vi "Layout.vi"(0 "reference":refnum<class "ClassRelationshipEdge.lvclass">, 1 "graph":refnum<class "Graph.lvclass">, 2 "graphics":refnum<class "Graphics.lvclass">, 3 "grid":refnum<class "Grid.lvclass">, 5 "error in (no error)":errorcluster) -> (14 "reference out":refnum<class "ClassRelationshipEdge.lvclass">, 19 "error out":errorcluster)   [LabVIEW 2020, in "ClassRelationshipEdge.lvclass"]
uses:
  <resource>/Framework/Providers/Open_GDS/UML/ClassRelationshipEdge_class/ClassRelationshipEdge.lvclass
  C:/Program Files (x86)/National Instruments/LabVIEW 2020/resource/Framework/Providers/Open_GDS/UML/AbstractEdge_class/AbstractEdge.lvclass
  <resource>/Framework/Providers/Open_GDS/UML/Grid_class/Grid.lvclass
  <resource>/Framework/Providers/Open_GDS/UML/Graphics_class/Graphics.lvclass
  <resource>/Framework/Providers/Open_GDS/UML/Graph_class/Graph.lvclass
  <resource>/Framework/Providers/Open_GDS/UML/BentStyle_class/BentStyle.lvclass
  <resource>/Framework/Providers/Open_GDS/UML/AbstractNode_class/AbstractNode.lvclass
  <resource>/Framework/Providers/Open_GDS/UML/AbstractEdge_class/AbstractEdge.lvclass
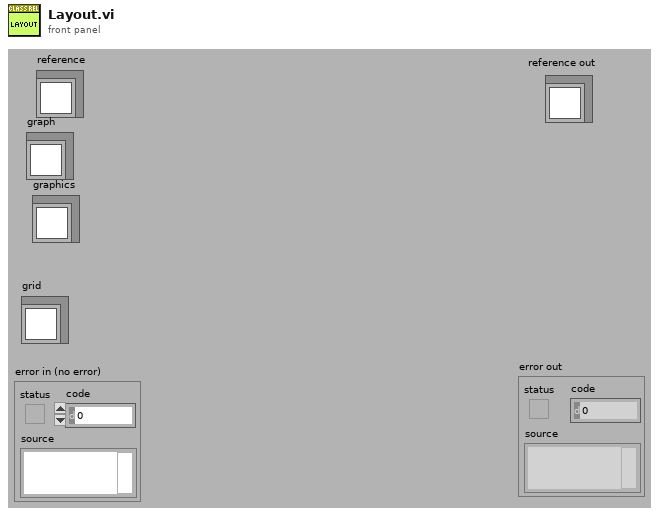
[diagram p1: front panel]
types:
  T1 = typedef "ClassRelationshipEdge.lvclass/ObjectAttributes.ctl" = cluster{"bentStyleRef":refnum<class "BentStyle.lvclass">, "startConnectionOffset":cluster{"x":i32, "y":i32}, "endConnectionOffset":cluster{"x":i32, "y":i32}, "MidLineOffset":cluster{"x":i32, "y":i32}, "DepClass":T2}
  T2 = typedef "ReversedEngineering_ViDependencyDetailsType.ctl" = cluster{"ThisVIs/Ctls":path[], "Dependent_VIs/Ctls":path[]}
  T3 = typedef "AbstractEdge.lvclass/ObjectAttributes.ctl" = cluster{"start":refnum<class "AbstractNode.lvclass">, "end":refnum<class "AbstractNode.lvclass">}
  T4 = typedef "Rectangle Rectangle2D.ctl" = cluster{"x":dbl, "y":dbl, "width":dbl, "height":dbl}
  T5 = typedef "Point Point2D.ctl" = cluster{"x":dbl, "y":dbl}
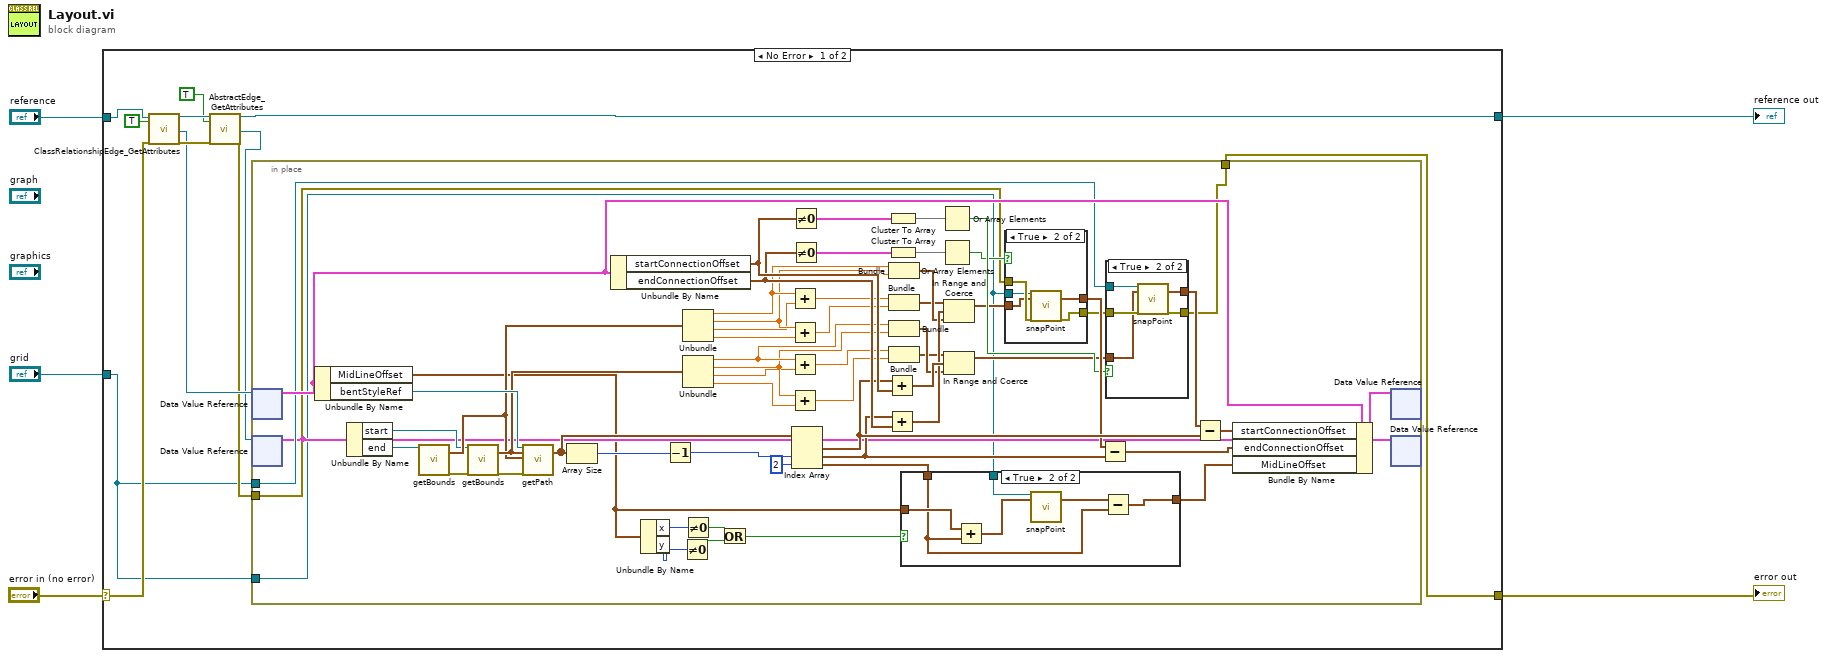
[diagram p0: block diagram]
diagram:
  n1 = case shown="No Error" "error in (no error)" {
    selector: "error in (no error)" -> [w17 w100]
    tunnel: "reference" -> [w16 w101]
    tunnel: [w15 w100] -> w3
    tunnel: [w14 w101] -> w2
    tunnel: "grid" -> [w7 _]
    frame No Error {
      n2 = call <resource>:"ClassRelationshipEdge_GetAttributes.vi"("reference in"=w16, "OnlyGetDvrReference(False)"=TRUE, "error in (no error)"=w17) -> ("reference out"=w12:refnum<class "ClassRelationshipEdge.lvclass">, "DataRef"=w10:refnum<data-value>, "error out"=w11:errorcluster)  [unwired: 13 in, 1 out]
      n3 = call <resource>:"AbstractEdge_GetAttributes.vi"("reference in"=w12, "OnlyGetDvrReference(False)"=TRUE, "error in (no error)"=w11) -> ("reference out"=w14:refnum<class "ClassRelationshipEdge.lvclass">, "DataRef"=w9:refnum<data-value>, "error out"=w8:errorcluster)  [unwired: 13 in, 1 out]
      n4 = in-place {
        in-place-border: w7 -> [w56]
        in-place-border: [w55] -> w15
        in-place-border: w8 -> [w53]
        in-place-border: w7 -> [w27]
        n5 = in-place-dvr #1(w10) -> (w78:T1)  [unwired: 1 out]
        n6 = in-place-dvr #2(w9) -> (w28:T3)  [unwired: 1 out]
        n7 = Unbundle By Name(w78) -> ("MidLineOffset"=w20:cluster{"x":i32, "y":i32}, "bentStyleRef"=w75:refnum<class "BentStyle.lvclass">)
        n8 = Unbundle By Name(w28) -> ("start"=w51:refnum<class "AbstractNode.lvclass">, "end"=w45:refnum<class "AbstractNode.lvclass">)
        n9 = call-dynamic "getBounds.vi"("reference"=w45) -> ("bounds"=w67:T4, "error out"=w50:errorcluster)  [unwired: 1 in, 16 out]
        n10 = call-dynamic "getBounds.vi"("reference"=w51, "error in (no error)"=w50) -> ("bounds"=w68:T4, "error out"=w66:errorcluster)  [unwired: 16 out]
        n11 = call-dynamic "getPath.vi"("reference"=w75, "start"=w68, "end"=w67, "error in (no error)"=w66) -> ("path"=w65:T5[])  [unwired: 15 out]
        n12 = Array Size(array=w65) -> (size(s)=w40:i32)
        n13 = Unbundle By Name(w78) -> ("startConnectionOffset"=w74:cluster{"x":i32, "y":i32}, "endConnectionOffset"=w73:cluster{"x":i32, "y":i32})
        n14 = Unbundle By Name(w20) -> ("x"=w24:i32, "y"=w23:i32)
        n15 = Decrement(x=w40) -> (x-1=w60:i32)
        n16 = Not Equal To 0?(x=w23) -> (x != 0?=w21:bool)
        n17 = Unbundle(w67) -> ("x"=w44:dbl, "y"=w43:dbl, "width"=w42:dbl, "height"=w41:dbl)
        n18 = Unbundle(w68) -> ("x"=w49:dbl, "y"=w48:dbl, "width"=w47:dbl, "height"=w46:dbl)
        n19 = Not Equal To 0?(x=w24) -> (x != 0?=w22:bool)
        n20 = Or(x=w22, y=w21) -> (x .or. y?=w18:bool)
        n21 = Add(x=w44, y=w42) -> (x+y=w31:dbl)
        n22 = Add(x=w43, y=w41) -> (x+y=w30:dbl)
        n23 = Add(x=w49, y=w47) -> (x+y=w33:dbl)
        n24 = Add(x=w48, y=w46) -> (x+y=w32:dbl)
        n25 = Not Equal To 0?(x=w74) -> (x != 0?=w64:cluster{"x":bool, "y":bool})
        n26 = Not Equal To 0?(x=w73) -> (x != 0?=w61:cluster{"x":bool, "y":bool})
        n27 = Index Array(array=w65, index #2=w60, index #3=2 ("index")) -> (element #1=w72:T5, element #2=w70:T5, element #3=w19:T5)  [unwired: 1 in]
        n28 = Add(x=w72, y=w74) -> (x+y=w63:T5)
        n29 = Add(x=w70, y=w73) -> (x+y=w62:T5)
        n30 = Cluster To Array(cluster=w64) -> (array=w39:bool[])
        n31 = Cluster To Array(cluster=w61) -> (array=w34:bool[])
        n32 = Bundle("x"=w44, "y"=w43) -> (w36:cluster{"x":dbl, "y":dbl})  [unwired: 1 out]
        n33 = Bundle(w31, w30) -> (w35:cluster{dbl, dbl})  [unwired: 1 out]
        n34 = Bundle("x"=w49, "y"=w48) -> (w38:cluster{"x":dbl, "y":dbl})  [unwired: 1 out]
        n35 = Bundle(w33, w32) -> (w37:cluster{dbl, dbl})  [unwired: 1 out]
        n36 = case shown="True" w18 {
          tunnel: w27 -> [_ w85]
          tunnel: [w79 w83] -> w25
          tunnel: w20 -> [w79 w82]
          tunnel: w19 -> [_ w80]
          frame False {
          }
          frame True {
            n37 = Add(x=w82, y=w80) -> (x+y=w81:T5)
            n38 = call <resource>:"snapPoint.vi"("reference"=w85, "point2D"=w81) -> ("point2D 2"=w84:T5)  [unwired: 1 in, 16 out]
            n39 = Subtract(x=w84, y=w80) -> (x-y=w83:T5)
          }
        }
        n40 = Or Array Elements(Boolean array=w39) -> (logical OR=w59:bool)
        n41 = Or Array Elements(Boolean array=w34) -> (logical OR=w54:bool)
        n42 = In Range and Coerce(upper limit=w35, x=w62, lower limit=w36) -> (coerced(x)=w52:T5)  [unwired: 1 out]
        n43 = In Range and Coerce(upper limit=w37, x=w63, lower limit=w38) -> (coerced(x)=w57:T5)  [unwired: 1 out]
        n44 = case shown="True" w54 {
          tunnel: w53 -> [w86 w92]
          tunnel: w27 -> [_ w91]
          tunnel: w52 -> [w87 w90]
          tunnel: [w87 w89] -> w69
          tunnel: [w86 w88] -> w58
          frame False {
          }
          frame True {
            n45 = call <resource>:"snapPoint.vi"("reference"=w91, "point2D"=w90, "error in (no error)"=w92) -> ("point2D 2"=w89:T5, "error out"=w88:errorcluster)  [unwired: 15 out]
          }
        }
        n46 = Subtract(x=w69, y=w70) -> (x-y=w76:T5)
        n47 = case shown="True" w59 {
          tunnel: w58 -> [w93 w99]
          tunnel: w57 -> [w94 w98]
          tunnel: [w94 w97] -> w71
          tunnel: w56 -> [_ w96]
          tunnel: [w93 w95] -> w55
          frame False {
          }
          frame True {
            n48 = call <resource>:"snapPoint.vi"("reference"=w96, "point2D"=w98, "error in (no error)"=w99) -> ("point2D 2"=w97:T5, "error out"=w95:errorcluster)  [unwired: 15 out]
          }
        }
        n49 = Subtract(x=w71, y=w72) -> (x-y=w77:T5)
        n50 = Bundle By Name(cluster=w78, "startConnectionOffset"=w77, "endConnectionOffset"=w76, "MidLineOffset"=w25) -> (w29:T1)
        n51 = in-place-dvr #1(w29) -> ()  [unwired: 2 out]
        n52 = in-place-dvr #2(w28) -> ()  [unwired: 2 out]
      }
    }
    frame Error {
    }
  }
  "reference out" <- w2
  "error out" <- w3
